vi "onTestDiscovery.vi"(8 "error in (no error)":errorcluster, 11 "Test Runner.Project in":refnum<class "Test Runner.Project.lvclass">) -> (0 "error out":errorcluster, 2 "Tests VIs":path[](array[path]), 3 "Test Runner.Project out":refnum<class "Test Runner.Project.lvclass">)   [LabVIEW 2020, in "Caraya.lvlib" / "Test Runner.Project.lvclass"]
uses:
  Test Runner.Project.lvclass
  C:/projects/caraya/src/classes/Test Runner/Test Runner.lvclass
  Test Runner.Project.lvclass/Test Runner.Project.ctl
  Test Runner/Test Runner.lvclass/Test Runner.ctl
  Test Runner/Test Runner.lvclass
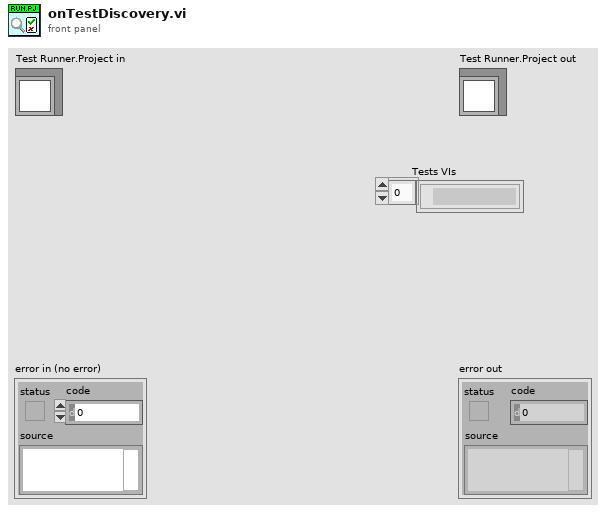
[diagram p1: front panel]
types:
  T1 = typedef "NI_FileType.lvlib/LVFileType.ctl" = enum32{"Invalid file", "Unknown type", "Instrument", "Control", "Polymorphic VI", "Project", "Library", "LVClass", "XControl", "XNode", "Shared library", ".NET assembly", "ActiveX interface", "CIN", "Run-time menu", "Palette menu", "Help file", "LLB", "XNode Edit Dependency", "Class Private Data Control", "Statechart", "MathScript .m file", "Ladder Diagram", "LVLibp", "XNode Build Dependency"}
  T2 = cluster{"path":path, "delimited name":string, "type":T1, "iState":u32, "iStyle":u16, "wStyle":u16, "buttons":u16, "viflags":u32, "viflags2":u32, "links":u32[]}[]
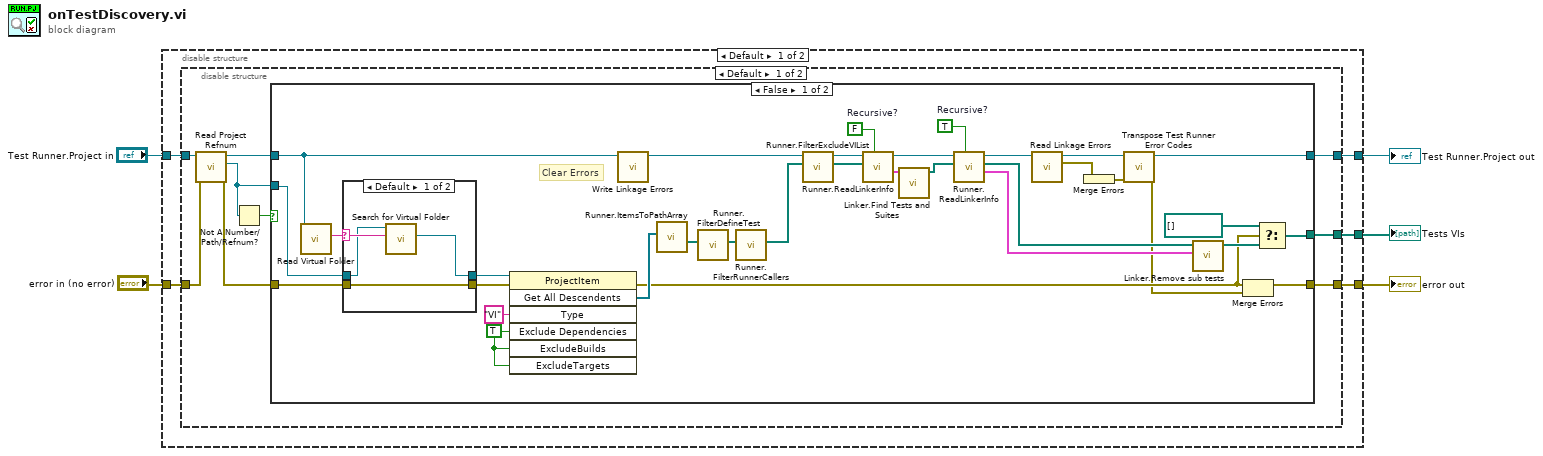
[diagram p0: block diagram]
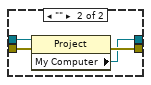
[diagram p2: hidden frame]
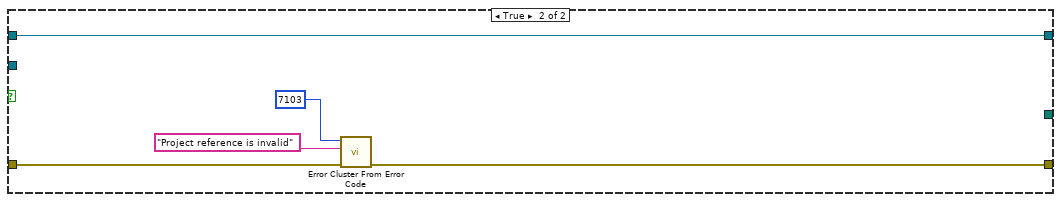
[diagram p3: hidden frame]
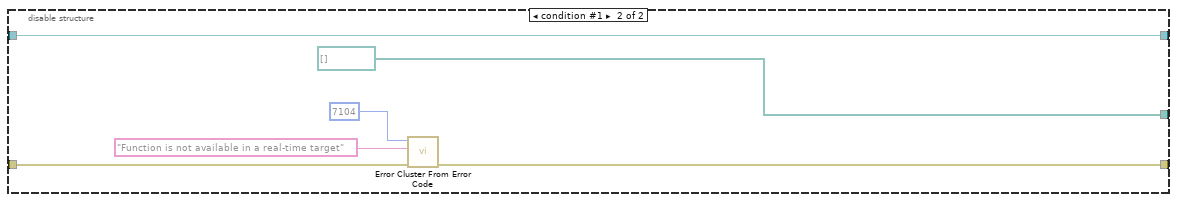
[diagram p4: hidden frame]
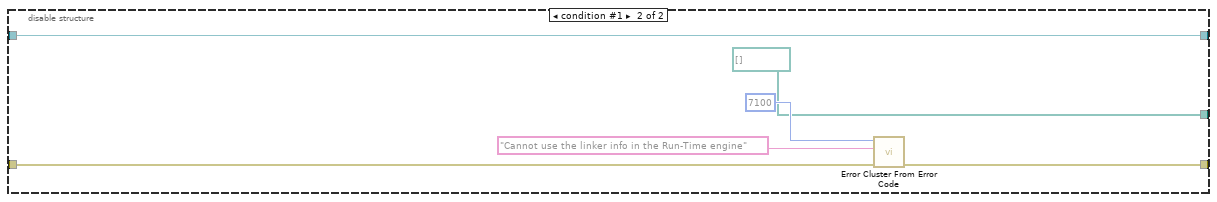
[diagram p5: hidden frame]
diagram:
  n1 = disable-structure shown="Default" {
    disable-tunnel: [w10 w75] -> w2
    disable-tunnel: "Test Runner.Project in" -> [w6 w74]
    disable-tunnel: [w9 w74] -> w3
    disable-tunnel: [w8 path[] [] ("Test VIs")] -> w1
    disable-tunnel: "error in (no error)" -> [w7 w72]
    frame condition #0 (active) {
      n2 = disable-structure shown="Default" {
        disable-tunnel: [w19 w67] -> w10
        disable-tunnel: [w18 w71] -> w9
        disable-tunnel: [w17 path[] [] ("Test VIs")] -> w8
        disable-tunnel: w7 -> [w15 w68]
        disable-tunnel: w6 -> [w13 w71]
        frame condition #0 (active) {
          n3 = call "Read Project Refnum.vi"("error in (no error)"=w15, "Test Runner.Project in"=w13) -> ("error out"=w14:errorcluster, "Project Refnum"=w11:refnum<vi>, "Test Runner.Project out"=w12:refnum<class "Test Runner.Project.lvclass">)  [unwired: 7 in]
          n4 = Not A Number/Path/Refnum?(number/path/refnum=w11) -> (NaN/Path/Refnum?=w16:bool)
          n5 = case shown="False" w16 {
            tunnel: [w30 w61] -> w19
            tunnel: [w52 _] -> w17
            tunnel: w11 -> [w45 _]
            tunnel: w12 -> [w39 w65]
            tunnel: [w25 w65] -> w18
            tunnel: w14 -> [w46 w62]
            frame False {
              w33 = FALSE  # Recursive?
              w32 = TRUE  # Recursive?
              w49 = TRUE ("ExcludeDependencies")
              # "Clear Errors"
              n6 = call "Read Virtual Folder.vi"("Test Runner.Project in"=w39) -> ("Virtual Folder"=w44:string)  [unwired: 9 in, 1 out]
              n7 = case shown="Default" w44 {
                selector: w44 -> [w56 _]
                tunnel: [w53 w60] -> w50
                tunnel: [w55 w57] -> w47
                tunnel: w46 -> [w53 w59]
                tunnel: w45 -> [w54 w58]
                frame Default {
                  n8 = call "Search for Virtual Folder.vi"("Virtual Folder"=w56, "Project Refnum"=w54) -> ("best match"=w55:refnum<vi>)  [unwired: 6 in, 3 out]
                }
                frame "" {
                  n9 = property class="Project"(reference=w58, error in=w59) -> (error out=w60:errorcluster, "My Computer"=w57:refnum<vi>)  [unwired: 1 out]
                }
              }
              n10 = invoke class="ProjectItem" method="Get All Descendents"(reference=w47, error in=w50, "Type"="VI", "Exclude Dependencies"=w49, "ExcludeBuilds"=w49, "ExcludeTargets"=w49) -> (error out=w31:errorcluster, "All Descendents"=w40:refnum<vi>[])  [unwired: 1 in, 5 out]
              n11 = call "Write Linkage Errors.vi"("Test Runner in"=w39) -> ("Test Runner out"=w23:refnum<class "Test Runner.Project.lvclass">)  [unwired: 9 in, 1 out]
              n12 = call "Runner.ItemsToPathArray.vi"("Project Items"=w40) -> ("Paths"=w42:path[])  [unwired: 10 in]
              n13 = call "Runner.FilterDefineTest.vi"("Paths"=w42) -> ("Filtered Paths"=w41:path[])  [unwired: 10 in]
              n14 = call "Runner.FilterRunnerCallers.vi"("Paths"=w41) -> ("Filtered Paths"=w21:path[])  [unwired: 10 in]
              n15 = call "Runner.FilterExcludeVIList.vi"("Paths"=w21, "Test Runner"=w23) -> ("Filtered Paths"=w20:path[], "Test Runner"=w22:refnum<class "Test Runner.Project.lvclass">)  [unwired: 8 in]
              n16 = call "Runner.ReadLinkerInfo.vi"("Recursive?"=w33, "VI Paths"=w20, "Test Runner in"=w22) -> ("Linker:Read Info From File"=w37:T2, "Test Runner out"=w38:refnum<class "Test Runner.Project.lvclass">)  [unwired: 5 in, 2 out]
              n17 = call "Linker.Find Tests and Suites.vi"("Linker:Read Info From File"=w37) -> ("All VIs defining a test (excluding those defining a suite)"=w35:path[])  [unwired: 8 in, 2 out]
              n18 = call "Runner.ReadLinkerInfo.vi"("Recursive?"=w32, "VI Paths"=w35, "Test Runner in"=w38) -> ("Linker:Read Info From File"=w36:T2, "VI Paths (dup)"=w34:path[], "Test Runner out"=w26:refnum<class "Test Runner.Project.lvclass">)  [unwired: 5 in, 1 out]
              n19 = call "Read Linkage Errors.vi"("Test Runner in"=w26) -> ("Linkage Errors"=w27:errorcluster[], "Test Runner out"=w29:refnum<class "Test Runner.Project.lvclass">)  [unwired: 8 in, 1 out]
              n20 = Merge Errors(w27) -> (w28:errorcluster)
              n21 = call-dynamic "Transpose Test Runner Error Codes.vi"("error in (no error)"=w28, "Test Runner in"=w29) -> ("error out"=w24:errorcluster, "Test Runner out"=w25:refnum<class "Test Runner.Project.lvclass">)  [unwired: 8 in]
              n22 = call "Linker.Remove sub tests.vi"("Linker.Read Info From File"=w36, "Tests"=w34) -> ("Array"=w43:path[])  [unwired: 9 in]
              n23 = Merge Errors(w31, w24) -> (w30:errorcluster)
              n24 = Select(t=path[] [], s=w31, f=w43) -> (s? t:f=w52:path[])
            }
            frame True {
              n25 = call <vilib>:"Error Cluster From Error Code.vi"("error in (no error)"=w62, "error message (\"\")"="Project reference is invalid" ("error message (\"\")"), "error code (0)"=7103) -> ("error out"=w61:errorcluster)  [unwired: 6 in]
            }
          }
        }
        frame condition #1 {
          n26 = call <vilib>:"Error Cluster From Error Code.vi"("error in (no error)"=w68, "error message (\"\")"="Function is not available in a real-time target" ("error message (\"\")"), "error code (0)"=7104) -> ("error out"=w67:errorcluster)  [unwired: 6 in]
        }
      }
    }
    frame condition #1 {
      n27 = call <vilib>:"Error Cluster From Error Code.vi"("error in (no error)"=w72, "error message (\"\")"="Cannot use the linker info in the Run-Time engine" ("error message (\"\")"), "error code (0)"=7100) -> ("error out"=w75:errorcluster)  [unwired: 6 in]
    }
  }
  "error out" <- w2
  "Test Runner.Project out" <- w3
  "Tests VIs" <- w1
